vi "GpuMat LocateROI.vi"(8 "error in (no error)":errorcluster, 11 "Src in":refnum<class "GpuMat.lvclass">) -> (0 "error out":errorcluster, 1 "WholeSize":T1, 2 "TopLeft":T1, 3 "Src out":refnum<class "GpuMat.lvclass">)   [LabVIEW 2020, in "OpenLvVision_OpenCv.lvlib" / "Cuda.lvlib" / "GpuMat.lvclass"]
doc: "Locates GpuMat header within a parent GpuMat."
uses:
  GpuMat.lvclass
  C:/Users/lukas/Documents/OpenLvVision_OpenCv/SourceCode/LabView/OpenLvVision_OpenCv/_LvHelpers/EdvrObject/EdvrObject.lvclass
  TypeDef/Point/2D_PointI32.ctl
  _LvHelpers/EdvrObject/EdvrObject.lvclass/EdvrObject.ctl
  OpenLvVision_OpenCv.lvlib
  <vilib>/Utility/error.llb/Error Cluster From Error Code.vi
  <vilib>/ErrorRing/Error Ring.xnode
  _LvHelpers/EdvrObject/EdvrObject.lvclass
  Dlls/OlvOpenCvWrapper.dll
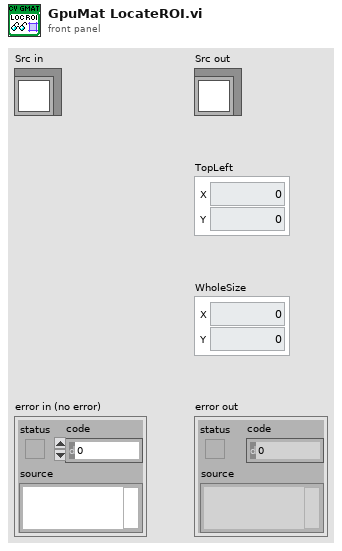
[diagram p1: front panel]
types:
  T1 = typedef "OpenLvVision_OpenCv.lvlib/2D_PointI32.ctl" = cluster{"X":i32, "Y":i32}
  T2 = typedef "OpenLvVision_OpenCv.lvlib/EdvrObject.lvclass/Edvr.ctl" = refnum<data-value>
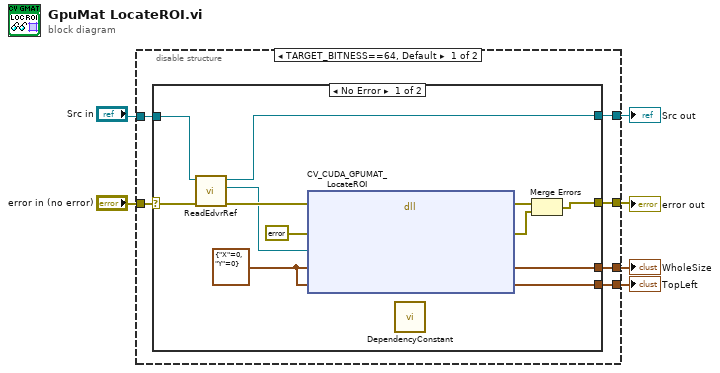
[diagram p0: block diagram]
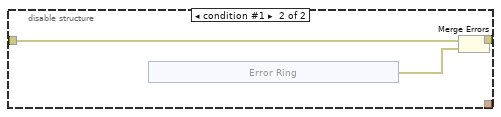
[diagram p3: hidden frame]
diagram:
  n1 = disable-structure shown="TARGET_BITNESS==64, Default" {
    disable-tunnel: "error in (no error)" -> [w12 w28]
    disable-tunnel: [w11 w29] -> w6
    disable-tunnel: "Src in" -> [w10 _]
    disable-tunnel: [w9 _] -> w3
    disable-tunnel: [w8 _] -> w2
    disable-tunnel: [w7 _] -> w1
    frame condition #0 (active) {
      n2 = case shown="No Error" w12 {
        selector: w12 -> [w17 w26]
        tunnel: [w16 w26] -> w11
        tunnel: w10 -> [w19 w25]
        tunnel: [w18 w25] -> w9
        tunnel: [w14 _] -> w8
        tunnel: [w13 _] -> w7
        frame No Error {
          w15 = T1 {"X"=0, "Y"=0} ("Point")
          n3 = call "ReadEdvrRef.vi"("error in (no error)"=w17, "EdvrObject in"=w19) -> ("error out"=w21:errorcluster, "Edvr"=w20:T2, "EdvrObject out"=w18:refnum<class "GpuMat.lvclass">)  [unwired: 7 in]
          n4 = dll-call lib="C:/Users/lukas/Documents/OpenLvVision_OpenCv/SourceCode/LabView/OpenLvVision_OpenCv/Dlls/OlvOpenCvWrapper.dll" fn="CV_CUDA_GPUMAT_LocateROI"(error in=w21, "Error"=errorcluster {"status"=FALSE, "code"=0, "source"=""} ("error out"), "srcRef"=w20, "wholeSize"=w15, "TopLeft"=w15) -> (error out=w24:errorcluster, "Error"=w23:errorcluster, "wholeSize"=w14:T1, "TopLeft"=w13:T1)  [unwired: 4 in, 1 out]
          n5 = call "DependencyConstant.vi"() -> ()  [unwired: 12 in]
          n6 = Merge Errors(w24, w23) -> (w16:errorcluster)
        }
        frame Error {
        }
      }
    }
    frame condition #1 {
      n7 = xnode "Error Ring"() -> ("error out"=w27:errorcluster)
      n8 = Merge Errors(w28, w27) -> (w29:errorcluster)
    }
  }
  "error out" <- w6
  "Src out" <- w3
  "WholeSize" <- w2
  "TopLeft" <- w1
